vi "Versioned Load.vi"(10 "path":path) -> (0 "Reversals":T10, 1 "Trajectory Data":T1, 2 "Zero V":bool, 3 "Commands out":cluster{"Time (s)":dbl, T8, bool}[](array[cluster]), 4 "Fields":T7 {"Overrides"."Angle Override" step=5.0; "Overrides"."Velocity Override" step=5.0; "Overrides"."Angular Override" step=5.0; "Angular Limits"."Jerk (deg/s^3)" min=0.0 step=1.0; "Angular Limits"."Accel (deg/s^2)" min=0.0; "Angular Limits"."Velocity (deg/s)" min=0.0}, 5 "Points out":cluster{"x":dbl, "y":dbl, "th":dbl}[](array[cluster]), 6 "Trajectory Meta":cluster{"Drive Type":T3, "Path Type":T4}, 7 "Overall":cluster{"Time (s)":dbl, "Distance (ft)":dbl})   [LabVIEW 2025]
uses:
  bordeaux-main/Bordeaux/Types/Single Cmd Info.ctl
  <vilib>/picture/picture.llb/imagedata.ctl
  bordeaux-main/Bordeaux/Types/Overrides.ctl
  bordeaux-main/Bordeaux/Types/Angluar Limits.ctl
  bordeaux-main/Bordeaux/Types/Drive Type.ctl
  bordeaux-main/Bordeaux/Types/Path Type.ctl
  bordeaux-main/Bordeaux/Types/Trajectory Data.ctl
  bordeaux-main/Bordeaux/Types/Segment Type.ctl
  bordeaux-main/Bordeaux/Types/Availible Command systems for auto.ctl
  bordeaux-main/Bordeaux/Types/Limits.ctl
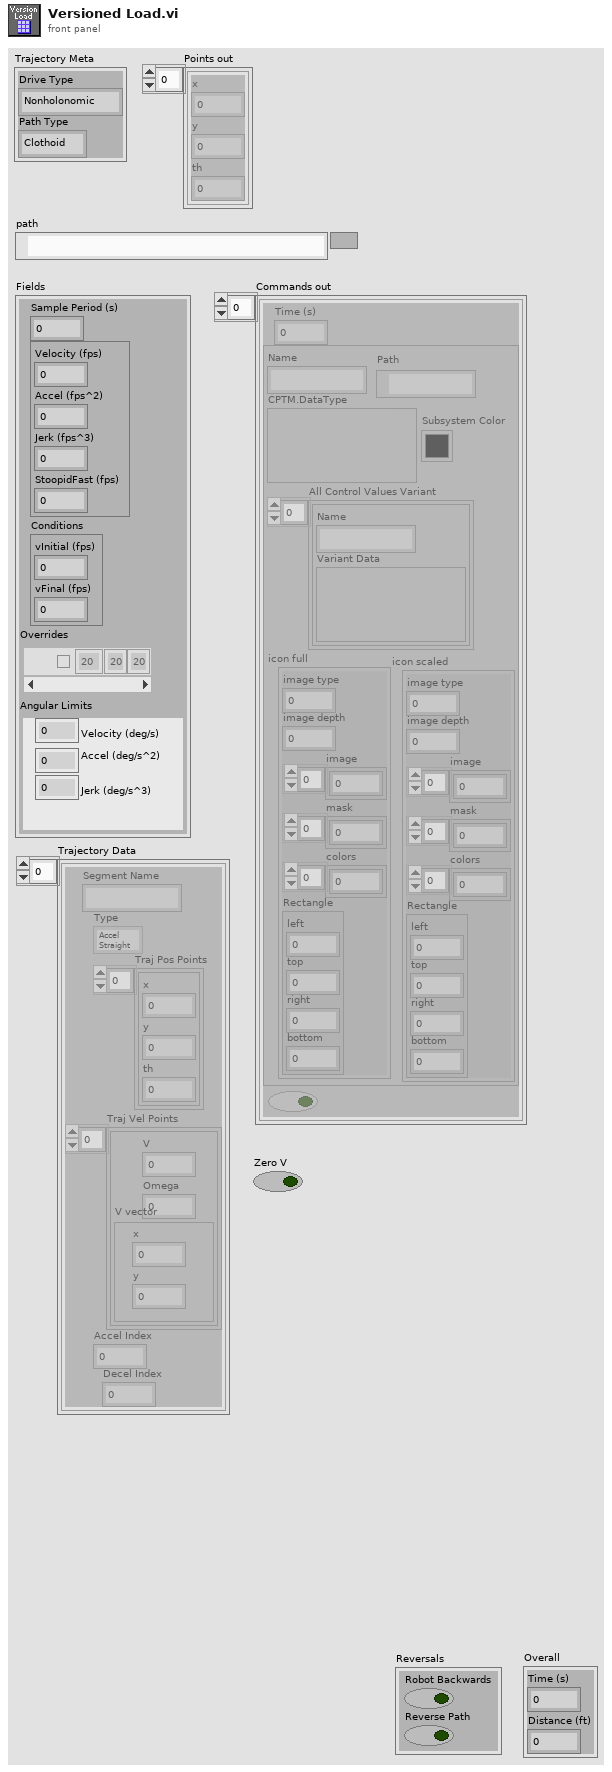
[diagram p1: front panel]
types:
  T1 = typedef "Trajectory Data.ctl" = cluster{"Segment Name":string, "Type":T2, "Traj Pos Points":cluster{"x":dbl, "y":dbl, "th":dbl}[], "Traj Vel Points":cluster{"V":dbl, "Omega":dbl, "V vector":cluster{"y":dbl, "x":dbl}}[], "Accel Index":i32, "Decel Index":i32}[]
  T2 = typedef "Segment Type.ctl" = enum16{"Accel Straight", "Const Straight", "Blend", "Circle", "Bezier"}
  T3 = typedef "Drive Type.ctl" = enum16{"Nonholonomic", "Holonomic"}
  T4 = typedef "Path Type.ctl" = enum16{"Clothoid", "Bezier"}
  T5 = typedef "Overrides.ctl" = cluster{"Count":string, "Angular Override":dbl, "Enabled?":bool, "Velocity Override":dbl, "Angle Override":dbl}[]
  T6 = typedef "Angluar Limits.ctl" = cluster{"Velocity (deg/s)":dbl, "Accel (deg/s^2)":dbl, "Jerk (deg/s^3)":dbl}
  T7 = cluster{"Sample Period (s)":dbl, cluster{"Velocity (fps)":dbl, "Accel (fps^2)":dbl, "Jerk (fps^3)":dbl, "StoopidFast (fps)":dbl}, "Conditions":cluster{"vInitial (fps)":dbl, "vFinal (fps)":dbl}, "Overrides":T5, "Angular Limits":T6}
  T8 = typedef "Single Cmd Info.ctl" = cluster{"Name":string, "CPTM.DataType":variant, "All Control Values Variant":cluster{"Name":string, "Variant Data":variant}[], "icon full":T9, "icon scaled":T9, "Path":path, "Subsystem Color":u32}
  T9 = typedef "imagedata.ctl" = cluster{"image type":i32, "image depth":i32, "image":u8[], "mask":u8[], "colors":u32[], "Rectangle":cluster{"left":i16, "top":i16, "right":i16, "bottom":i16}}
  T10 = cluster{"Robot Backwards":bool, "Reverse Path":bool}
  T11 = cluster{"Sample Period (s)":dbl, "Limits 2":cluster{"Velocity (fps)":dbl, "Acceleration (fps^2)":dbl, "Jerk (fps^3)":dbl}, "Conditions":cluster{"vInitial (fps)":dbl, "vFinal (fps)":dbl}, " Acceleration Overrides":cluster{"Angular \nAccelerations":dbl[], "Accel Override Bools":bool[]}}
  T12 = cluster{"Velocity":dbl, "Sample Time":dbl, "Accel":dbl}
  T13 = cluster{"Sample Period (s)":dbl, "Limits":cluster{"Velocity (fps)":dbl, "Acceleration (fps^2)":dbl, "Jerk (fps^3)":dbl}, "Conditions":cluster{"vInitial (fps)":dbl, "vFinal (fps)":dbl}}
  T14 = cluster{"Sample Period (s)":dbl, "Limits":cluster{"Velocity (fps)":dbl, "Acceleration (fps^2)":dbl, "Jerk (fps^3)":dbl}, "Conditions":cluster{"vInitial (fps)":dbl, "vFinal (fps)":dbl}, "Min Rads":dbl[]}
  T15 = typedef "Availible Command systems for auto.ctl" = u16
  T16 = cluster{"Time into Path":dbl, "System":T15, "Item Selected?":bool, "System Selection":T15}[]
  T17 = cluster{"Sample Period (s)":dbl, "Limits 2":cluster{"Velocity (fps)":dbl, "Acceleration (fps^2)":dbl, "Jerk (fps^3)":dbl, "Stoopid Fast":dbl}, "Conditions":cluster{"vInitial (fps)":dbl, "vFinal (fps)":dbl}, " Acceleration Overrides":cluster{"Angular \nAccelerations":dbl[], "Accel Override Bools":bool[]}}
  T18 = cluster{"Sample Period (s)":dbl, "Limits":cluster{"Velocity (fps)":dbl, "Accel (fps^2)":dbl, "Turn Accel (fps^2)":dbl, "Jerk (fps^3)":dbl}, "Conditions":cluster{"vInitial (fps)":dbl, "vFinal (fps)":dbl}, cluster{dbl[], bool[]}}
  T19 = cluster{"Reverse Path":bool, "Robot Backwards":bool}
  T20 = typedef "Limits.ctl" = cluster{"Velocity (fps)":dbl, "Accel (fps^2)":dbl, "Jerk (fps^3)":dbl, "StoopidFast (fps)":dbl}
  T21 = cluster{"Sample Period (s)":dbl, "Limits":T20, "Conditions":cluster{"vInitial (fps)":dbl, "vFinal (fps)":dbl}, "Overrides":T5, "Angular Limits":T6}
  T22 = cluster{"Velocity":dbl, "Accel":dbl, "Accel":dbl, "Velocity":dbl}
  T23 = cluster{"Velocity (fps)":dbl, "Acceleration (fps^2)":dbl, "Jerk (fps^3)":dbl}
  T24 = cluster{"vInitial (fps)":dbl, "vFinal (fps)":dbl}
  T25 = cluster{"Velocity (fps)":dbl, "Acceleration (fps^2)":dbl, "Jerk (fps^3)":dbl, "Velocity (fps)":dbl}
  T26 = cluster{string, "Angular Multiplier":dbl, bool, "Velocity (fps)":dbl, "Velocity (fps)":dbl}
  T27 = cluster{"Angular \nAccelerations":dbl[], "Accel Override Bools":bool[]}
  T28 = cluster{"Velocity (fps)":dbl, "Acceleration (fps^2)":dbl, "Jerk (fps^3)":dbl, "Stoopid Fast":dbl}
  T29 = cluster{"Velocity (fps)":dbl, "Accel (fps^2)":dbl, "Turn Accel (fps^2)":dbl, "Jerk (fps^3)":dbl}
  T30 = cluster{"Velocity (fps)":dbl, "Accel (fps^2)":dbl, "Jerk (fps^3)":dbl, "StoopidFast (fps)":dbl}
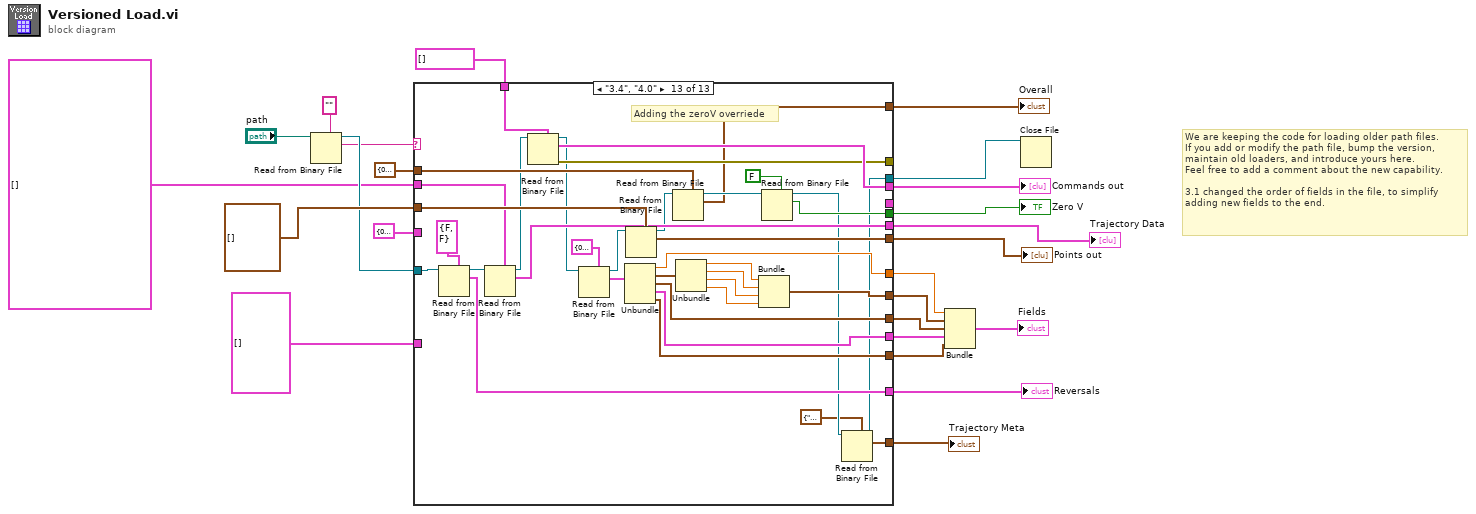
[diagram p0: block diagram]
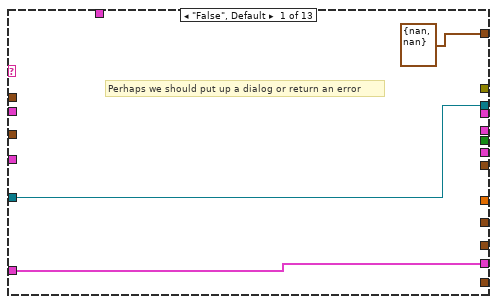
[diagram p2: hidden frame]
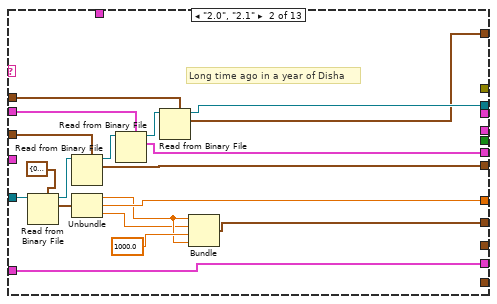
[diagram p3: hidden frame]
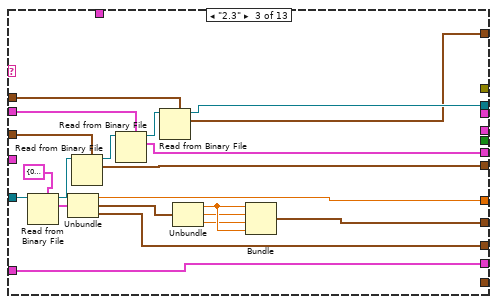
[diagram p4: hidden frame]
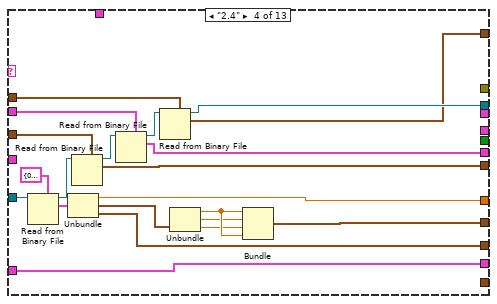
[diagram p5: hidden frame]
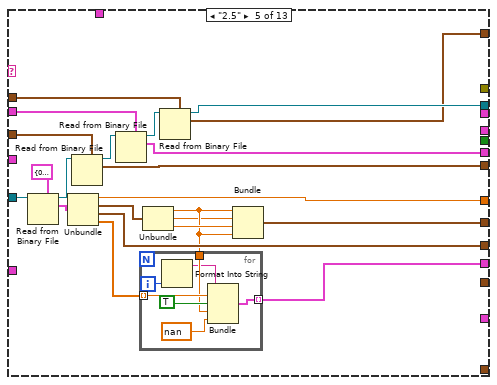
[diagram p6: hidden frame]
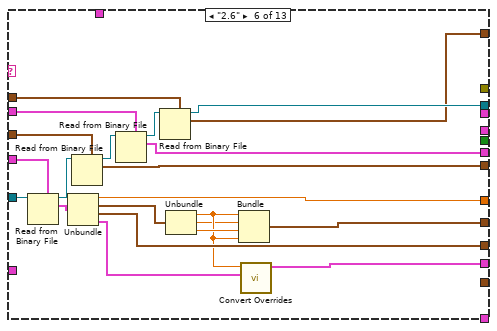
[diagram p7: hidden frame]
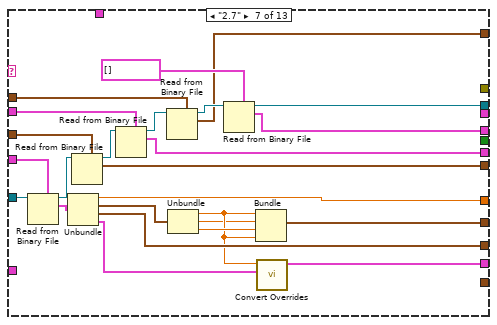
[diagram p8: hidden frame]
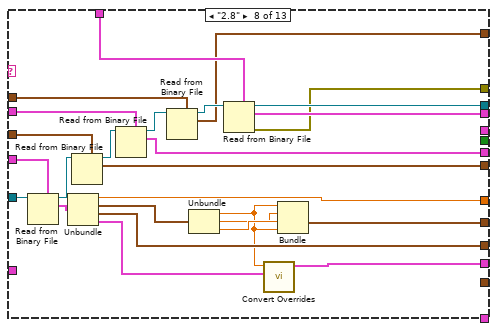
[diagram p9: hidden frame]
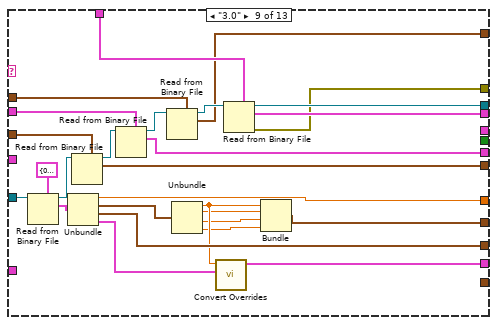
[diagram p10: hidden frame]
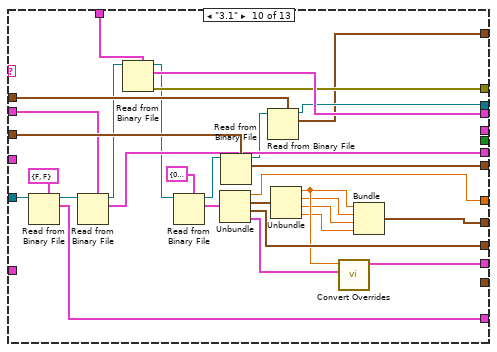
[diagram p11: hidden frame]
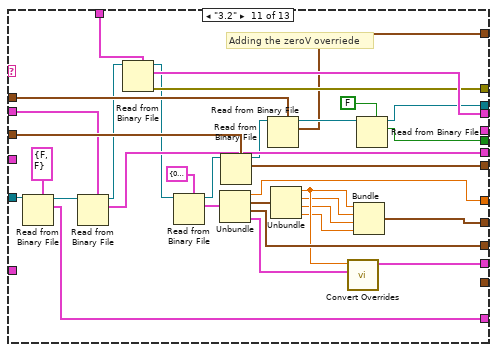
[diagram p12: hidden frame]
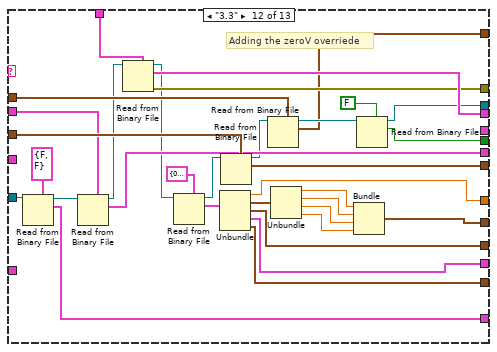
[diagram p13: hidden frame]
diagram:
  # "We are keeping the code for loading older path files.\nIf you add or modify the path file, bump the version,\nmaintain old loaders, and introduce yours here.\nFeel free to add a comment about the new capability.\n\n3.1 changed the order of fields in the file, to simplify\nadding new fields to the end."
  n1 = Read from Binary File(5:"" ("String"), 11:"path") -> (2:w7:string, 3:w8:refnum<file>)  [unwired: 4 in, 2 out]
  n2 = case shown="\"3.4\", \"4.0\"" w7 {
    tunnel: w8 -> [w27 w45 w66 w87 w109 w138 w163 w189 w216 w236 w269 w302 w338]
    tunnel: cluster{"x":dbl, "y":dbl, "th":dbl}[] [] ("Points in") -> [_ w43 w64 w85 w107 w136 w161 w187 w214 w245 w278 w311 w347]
    tunnel: [_ w42 w63 w84 w106 w135 w160 w186 w213 w244 w277 w310 w346] -> w14
    tunnel: T1 [] ("Trajectory Data") -> [_ w41 w62 w83 w105 w134 w159 w185 w212 w243 w276 w309 w345]
    tunnel: cluster{"Time (s)":dbl, "Distance (ft)":dbl} {"Time (s)"=0.0, "Distance (ft)"=0.0} ("Cluster 4") -> [_ w39 w60 w81 w103 w132 w157 w183 w210 w242 w275 w308 w344]
    tunnel: [w27 w37 w58 w79 w101 w130 w151 w177 w204 w232 w251 w287 w315] -> w10
    tunnel: [_ w35 w57 w78 w100 w129 w155 w181 w208 w219 w253 w289 w325] -> w21
    tunnel: [_ w31 w51 w71 w94 w124 w145 w172 w192 w224 w258 w294 w330] -> w22
    tunnel: [_ _ w56 w77 w99 w128 w154 w180 w207 w241 w274 w307 w343] -> w23
    tunnel: [w26 w30 w50 w70 w93 w122 w142 w169 w198 w228 w262 w282 w319] -> w24
    tunnel: [_ w33 w54 w75 w97 w127 w153 w179 w206 w240 w273 w306 w342] -> w13
    tunnel: [_ _ _ _ _ _ w150 _ _ _ _ _ _] -> _
    tunnel: cluster{"Time (s)":dbl, T8, bool}[] [] ("Commands in") -> [_ _ _ _ _ _ _ w176 w203 w239 w272 w305 w341]
    tunnel: [_ _ _ _ _ _ _ w175 w202 w238 w271 w304 w340] -> w16
    tunnel: [_ _ _ _ _ _ _ w174 w201 w237 w270 w303 w339] -> _
    tunnel: T11 {"Sample Period (s)"=0.0, "Limits 2"={"Velocity (fps)"=0.0, "Acceleration (fps^2)"=0.0, "Jerk (fps^3)"=0.0}, "Conditions"={"vInitial (fps)"=0.0, "vFinal (fps)"=0.0}, " Acceleration Overrides"={"Angular \nAccelerations"=[], "Accel Override Bools"=[]}} ("Cluster") -> [_ _ _ _ _ w126 w148 w170 _ _ _ _ _]
    tunnel: [_ _ _ _ _ _ _ _ _ w227 w261 w296 w332] -> w18
    tunnel: T5 [] ("Overrides") -> [w26 w30 w50 w70 _ _ _ _ _ _ _ _ _]
    tunnel: [_ _ _ _ _ _ _ _ _ _ w249 w285 w322] -> w19
    tunnel: [cluster{"Time (s)":dbl, "Distance (ft)":dbl} {"Time (s)"=nan, "Distance (ft)"=nan} ("Cluster 4") w28 w47 w68 w89 w118 w140 w165 w191 w218 w248 w284 w321] -> w5
    tunnel: [_ _ _ _ _ _ _ _ _ _ _ w281 w318] -> w2
    tunnel: [_ _ _ _ _ _ _ _ _ _ _ _ w314] -> w1
    frame "False", Default {
      # "Perhaps we should put up a dialog or return an error"
    }
    frame "2.0", "2.1" {
      # "Long time ago in a year of Disha"
      n3 = Read from Binary File(5:T12 {"Velocity"=0.0, "Sample Time"=0.0, "Accel"=0.0}, 11:w45) -> (2:w46:T12, 3:w44:refnum<file>)  [unwired: 4 in, 2 out]
      n4 = Read from Binary File(5:w43, 11:w44) -> (2:w42:cluster{"x":dbl, "y":dbl, "th":dbl}[], 3:w40:refnum<file>)  [unwired: 4 in, 2 out]
      n5 = Unbundle(w46) -> ("Velocity"=w32:dbl, "Sample Time"=w35:dbl, "Accel"=w29:dbl)
      n6 = Read from Binary File(5:w41, 11:w40) -> (2:w33:T1, 3:w38:refnum<file>)  [unwired: 4 in, 2 out]
      n7 = Read from Binary File(5:w39, 11:w38) -> (2:w28:cluster{"Time (s)":dbl, "Distance (ft)":dbl}, 3:w37:refnum<file>)  [unwired: 4 in, 2 out]
      n8 = Bundle("Velocity"=w32, "Accel"=w29, "Accel"=1000.0, "Velocity"=w32) -> (w31:T22)  [unwired: 1 in]
    }
    frame "2.3" {
      n9 = Read from Binary File(5:T13 {"Sample Period (s)"=0.0, "Limits"={"Velocity (fps)"=0.0, "Acceleration (fps^2)"=0.0, "Jerk (fps^3)"=0.0}, "Conditions"={"vInitial (fps)"=0.0, "vFinal (fps)"=0.0}}, 11:w66) -> (2:w67:T13, 3:w65:refnum<file>)  [unwired: 4 in, 2 out]
      n10 = Unbundle(w67) -> ("Sample Period (s)"=w57:dbl, "Limits"=w48:T23, "Conditions"=w56:T24)
      n11 = Read from Binary File(5:w64, 11:w65) -> (2:w63:cluster{"x":dbl, "y":dbl, "th":dbl}[], 3:w61:refnum<file>)  [unwired: 4 in, 2 out]
      n12 = Read from Binary File(5:w62, 11:w61) -> (2:w54:T1, 3:w59:refnum<file>)  [unwired: 4 in, 2 out]
      n13 = Read from Binary File(5:w60, 11:w59) -> (2:w47:cluster{"Time (s)":dbl, "Distance (ft)":dbl}, 3:w58:refnum<file>)  [unwired: 4 in, 2 out]
      n14 = Unbundle(w48) -> ("Velocity (fps)"=w53:dbl, "Acceleration (fps^2)"=w49:dbl, "Jerk (fps^3)"=w52:dbl)
      n15 = Bundle("Velocity (fps)"=w53, "Acceleration (fps^2)"=w49, "Jerk (fps^3)"=w52, "Velocity (fps)"=w53) -> (w51:T25)  [unwired: 1 in]
    }
    frame "2.4" {
      n16 = Read from Binary File(5:T13 {"Sample Period (s)"=0.0, "Limits"={"Velocity (fps)"=0.0, "Acceleration (fps^2)"=0.0, "Jerk (fps^3)"=0.0}, "Conditions"={"vInitial (fps)"=0.0, "vFinal (fps)"=0.0}}, 11:w87) -> (2:w88:T13, 3:w86:refnum<file>)  [unwired: 4 in, 2 out]
      n17 = Unbundle(w88) -> ("Sample Period (s)"=w78:dbl, "Limits"=w72:T23, "Conditions"=w77:T24)
      n18 = Read from Binary File(5:w85, 11:w86) -> (2:w84:cluster{"x":dbl, "y":dbl, "th":dbl}[], 3:w82:refnum<file>)  [unwired: 4 in, 2 out]
      n19 = Read from Binary File(5:w83, 11:w82) -> (2:w75:T1, 3:w80:refnum<file>)  [unwired: 4 in, 2 out]
      n20 = Read from Binary File(5:w81, 11:w80) -> (2:w68:cluster{"Time (s)":dbl, "Distance (ft)":dbl}, 3:w79:refnum<file>)  [unwired: 4 in, 2 out]
      n21 = Unbundle(w72) -> ("Velocity (fps)"=w74:dbl, "Acceleration (fps^2)"=w69:dbl, "Jerk (fps^3)"=w73:dbl)
      n22 = Bundle("Velocity (fps)"=w74, "Acceleration (fps^2)"=w69, "Jerk (fps^3)"=w73, "Velocity (fps)"=w74) -> (w71:T25)  [unwired: 1 in]
    }
    frame "2.5" {
      n23 = Read from Binary File(5:T14 {"Sample Period (s)"=0.0, "Limits"={"Velocity (fps)"=0.0, "Acceleration (fps^2)"=0.0, "Jerk (fps^3)"=0.0}, "Conditions"={"vInitial (fps)"=0.0, "vFinal (fps)"=0.0}, "Min Rads"=[20.0, 20.0, 20.0, 20.0, 20.0]}, 11:w109) -> (2:w110:T14, 3:w108:refnum<file>)  [unwired: 4 in, 2 out]
      n24 = Unbundle(w110) -> ("Sample Period (s)"=w100:dbl, "Limits"=w95:T23, "Conditions"=w99:T24, "Min Rads"=w92:dbl[])
      n25 = Read from Binary File(5:w107, 11:w108) -> (2:w106:cluster{"x":dbl, "y":dbl, "th":dbl}[], 3:w104:refnum<file>)  [unwired: 4 in, 2 out]
      n26 = Read from Binary File(5:w105, 11:w104) -> (2:w97:T1, 3:w102:refnum<file>)  [unwired: 4 in, 2 out]
      n27 = Unbundle(w95) -> ("Velocity (fps)"=w91:dbl, "Acceleration (fps^2)"=w90:dbl, "Jerk (fps^3)"=w96:dbl)
      n28 = for {
        tunnel: [w116] -> w93 mode=indexing
        tunnel: w92 -> [w115] mode=indexing
        tunnel: w91 -> [w114]
        i -> [w113]
        n29 = Format Into String(w113) -> (resulting string=w112:string)  [unwired: 3 in, 1 out]
        n30 = Bundle(w112, "Angular Multiplier"=w115, TRUE, "Velocity (fps)"=w114, "Velocity (fps)"=nan) -> (w116:T26)  [unwired: 1 in]
      }
      n31 = Read from Binary File(5:w103, 11:w102) -> (2:w89:cluster{"Time (s)":dbl, "Distance (ft)":dbl}, 3:w101:refnum<file>)  [unwired: 4 in, 2 out]
      n32 = Bundle("Velocity (fps)"=w91, "Acceleration (fps^2)"=w90, "Jerk (fps^3)"=w96, "Velocity (fps)"=w91) -> (w94:T25)  [unwired: 1 in]
    }
    frame "2.6" {
      n33 = Read from Binary File(5:w126, 11:w138) -> (2:w139:T11, 3:w137:refnum<file>)  [unwired: 4 in, 2 out]
      n34 = Unbundle(w139) -> ("Sample Period (s)"=w129:dbl, "Limits 2"=w123:T23, "Conditions"=w128:T24, "Acceleration Overrides"=w120:T27)
      n35 = Read from Binary File(5:w136, 11:w137) -> (2:w135:cluster{"x":dbl, "y":dbl, "th":dbl}[], 3:w133:refnum<file>)  [unwired: 4 in, 2 out]
      n36 = Read from Binary File(5:w134, 11:w133) -> (2:w127:T1, 3:w131:refnum<file>)  [unwired: 4 in, 2 out]
      n37 = Read from Binary File(5:w132, 11:w131) -> (2:w118:cluster{"Time (s)":dbl, "Distance (ft)":dbl}, 3:w130:refnum<file>)  [unwired: 4 in, 2 out]
      n38 = Unbundle(w123) -> ("Velocity (fps)"=w121:dbl, "Acceleration (fps^2)"=w119:dbl, "Jerk (fps^3)"=w125:dbl)
      n39 = Bundle("Velocity (fps)"=w121, "Acceleration (fps^2)"=w119, "Jerk (fps^3)"=w125, "Velocity (fps)"=w121) -> (w124:T25)  [unwired: 1 in]
      n40 = call "Convert Overrides.vi"("Cluster"=w120, "Velocity (fps)"=w121) -> ("Overrides"=w122:T5)  [unwired: 9 in]
    }
    frame "2.7" {
      n41 = Read from Binary File(5:w148, 11:w163) -> (2:w164:T11, 3:w162:refnum<file>)  [unwired: 4 in, 2 out]
      n42 = Unbundle(w164) -> ("Sample Period (s)"=w155:dbl, "Limits 2"=w146:T23, "Conditions"=w154:T24, "Acceleration Overrides"=w143:T27)
      n43 = Read from Binary File(5:w161, 11:w162) -> (2:w160:cluster{"x":dbl, "y":dbl, "th":dbl}[], 3:w158:refnum<file>)  [unwired: 4 in, 2 out]
      n44 = Read from Binary File(5:w159, 11:w158) -> (2:w153:T1, 3:w156:refnum<file>)  [unwired: 4 in, 2 out]
      n45 = Read from Binary File(5:w157, 11:w156) -> (2:w140:cluster{"Time (s)":dbl, "Distance (ft)":dbl}, 3:w152:refnum<file>)  [unwired: 4 in, 2 out]
      n46 = Unbundle(w146) -> ("Velocity (fps)"=w144:dbl, "Acceleration (fps^2)"=w141:dbl, "Jerk (fps^3)"=w147:dbl)
      n47 = Read from Binary File(5:T16 [] ("Commands"), 11:w152) -> (2:w150:T16, 3:w151:refnum<file>)  [unwired: 4 in, 2 out]
      n48 = Bundle("Velocity (fps)"=w144, "Acceleration (fps^2)"=w141, "Jerk (fps^3)"=w147, "Velocity (fps)"=w144) -> (w145:T25)  [unwired: 1 in]
      n49 = call "Convert Overrides.vi"("Cluster"=w143, "Velocity (fps)"=w144) -> ("Overrides"=w142:T5)  [unwired: 9 in]
    }
    frame "2.8" {
      n50 = Read from Binary File(5:w170, 11:w189) -> (2:w190:T11, 3:w188:refnum<file>)  [unwired: 4 in, 2 out]
      n51 = Unbundle(w190) -> ("Sample Period (s)"=w181:dbl, "Limits 2"=w173:T23, "Conditions"=w180:T24, "Acceleration Overrides"=w167:T27)
      n52 = Read from Binary File(5:w187, 11:w188) -> (2:w186:cluster{"x":dbl, "y":dbl, "th":dbl}[], 3:w184:refnum<file>)  [unwired: 4 in, 2 out]
      n53 = Read from Binary File(5:w185, 11:w184) -> (2:w179:T1, 3:w182:refnum<file>)  [unwired: 4 in, 2 out]
      n54 = Read from Binary File(5:w183, 11:w182) -> (2:w165:cluster{"Time (s)":dbl, "Distance (ft)":dbl}, 3:w178:refnum<file>)  [unwired: 4 in, 2 out]
      n55 = Unbundle(w173) -> ("Velocity (fps)"=w168:dbl, "Acceleration (fps^2)"=w166:dbl, "Jerk (fps^3)"=w171:dbl)
      n56 = Read from Binary File(5:w176, 11:w178) -> (0:w174:errorcluster, 2:w175:cluster{"Time (s)":dbl, T8, bool}[], 3:w177:refnum<file>)  [unwired: 4 in, 1 out]
      n57 = call "Convert Overrides.vi"("Cluster"=w167, "Velocity (fps)"=w168) -> ("Overrides"=w169:T5)  [unwired: 9 in]
      n58 = Bundle("Velocity (fps)"=w168, "Acceleration (fps^2)"=w166, "Jerk (fps^3)"=w171, "Velocity (fps)"=w168) -> (w172:T25)  [unwired: 1 in]
    }
    frame "3.0" {
      n59 = Read from Binary File(5:T17 {"Sample Period (s)"=0.0, "Limits 2"={"Velocity (fps)"=0.0, "Acceleration (fps^2)"=0.0, "Jerk (fps^3)"=0.0, "Stoopid Fast"=0.0}, "Conditions"={"vInitial (fps)"=0.0, "vFinal (fps)"=0.0}, " Acceleration Overrides"={"Angular \nAccelerations"=[], "Accel Override Bools"=[]}} ("Cluster"), 11:w216) -> (2:w217:T17, 3:w215:refnum<file>)  [unwired: 4 in, 2 out]
      n60 = Unbundle(w217) -> ("Sample Period (s)"=w208:dbl, "Limits 2"=w193:T28, "Conditions"=w207:T24, "Acceleration Overrides"=w199:T27)
      n61 = Read from Binary File(5:w214, 11:w215) -> (2:w213:cluster{"x":dbl, "y":dbl, "th":dbl}[], 3:w211:refnum<file>)  [unwired: 4 in, 2 out]
      n62 = Read from Binary File(5:w212, 11:w211) -> (2:w206:T1, 3:w209:refnum<file>)  [unwired: 4 in, 2 out]
      n63 = Read from Binary File(5:w210, 11:w209) -> (2:w191:cluster{"Time (s)":dbl, "Distance (ft)":dbl}, 3:w205:refnum<file>)  [unwired: 4 in, 2 out]
      n64 = Unbundle(w193) -> ("Velocity (fps)"=w197:dbl, "Acceleration (fps^2)"=w196:dbl, "Jerk (fps^3)"=w195:dbl, "Stoopid Fast"=w194:dbl)
      n65 = call "Convert Overrides.vi"("Cluster"=w199, "Velocity (fps)"=w197) -> ("Overrides"=w198:T5)  [unwired: 9 in]
      n66 = Read from Binary File(5:w203, 11:w205) -> (0:w201:errorcluster, 2:w202:cluster{"Time (s)":dbl, T8, bool}[], 3:w204:refnum<file>)  [unwired: 4 in, 1 out]
      n67 = Bundle("Velocity (fps)"=w197, "Acceleration (fps^2)"=w196, "Jerk (fps^3)"=w195, "Stoopid Fast"=w194) -> (w192:T28)  [unwired: 1 in]
    }
    frame "3.1" {
      n68 = Read from Binary File(5:T19 {"Reverse Path"=FALSE, "Robot Backwards"=FALSE} ("Cluster"), 11:w236) -> (2:w227:T19, 3:w233:refnum<file>)  [unwired: 4 in, 2 out]
      n69 = Read from Binary File(5:w243, 11:w233) -> (2:w240:T1, 3:w231:refnum<file>)  [unwired: 4 in, 2 out]
      n70 = Read from Binary File(5:w239, 11:w231) -> (0:w237:errorcluster, 2:w238:cluster{"Time (s)":dbl, T8, bool}[], 3:w230:refnum<file>)  [unwired: 4 in, 1 out]
      n71 = Read from Binary File(5:T18 {"Sample Period (s)"=0.0, "Limits"={"Velocity (fps)"=0.0, "Accel (fps^2)"=0.0, "Turn Accel (fps^2)"=15.0, "Jerk (fps^3)"=0.0}, "Conditions"={"vInitial (fps)"=0.0, "vFinal (fps)"=0.0}, {[], []}} ("Cluster 2"), 11:w230) -> (2:w247:T18, 3:w246:refnum<file>)  [unwired: 4 in, 2 out]
      n72 = Unbundle(w247) -> ("Sample Period (s)"=w219:dbl, "Limits"=w226:T29, "Conditions"=w241:T24, w229:cluster{dbl[], bool[]})
      n73 = Read from Binary File(5:w245, 11:w246) -> (2:w244:cluster{"x":dbl, "y":dbl, "th":dbl}[], 3:w234:refnum<file>)  [unwired: 4 in, 2 out]
      n74 = Read from Binary File(5:w242, 11:w234) -> (2:w218:cluster{"Time (s)":dbl, "Distance (ft)":dbl}, 3:w232:refnum<file>)  [unwired: 4 in, 2 out]
      n75 = Unbundle(w226) -> ("Velocity (fps)"=w223:dbl, "Accel (fps^2)"=w222:dbl, "Turn Accel (fps^2)"=w221:dbl, "Jerk (fps^3)"=w220:dbl)
      n76 = call "Convert Overrides.vi"("Cluster"=w229, "Velocity (fps)"=w223) -> ("Overrides"=w228:T5)  [unwired: 9 in]
      n77 = Bundle("Velocity (fps)"=w223, "Accel (fps^2)"=w222, "Turn Accel (fps^2)"=w221, "Jerk (fps^3)"=w220) -> (w224:T29)  [unwired: 1 in]
    }
    frame "3.2" {
      # "Adding the zeroV overriede"
      n78 = Read from Binary File(5:T10 {"Robot Backwards"=FALSE, "Reverse Path"=FALSE} ("Cluster"), 11:w269) -> (2:w261:T10, 3:w266:refnum<file>)  [unwired: 4 in, 2 out]
      n79 = Read from Binary File(5:w276, 11:w266) -> (2:w273:T1, 3:w265:refnum<file>)  [unwired: 4 in, 2 out]
      n80 = Read from Binary File(5:w272, 11:w265) -> (0:w270:errorcluster, 2:w271:cluster{"Time (s)":dbl, T8, bool}[], 3:w264:refnum<file>)  [unwired: 4 in, 1 out]
      n81 = Read from Binary File(5:T18 {"Sample Period (s)"=0.0, "Limits"={"Velocity (fps)"=0.0, "Accel (fps^2)"=0.0, "Turn Accel (fps^2)"=15.0, "Jerk (fps^3)"=0.0}, "Conditions"={"vInitial (fps)"=0.0, "vFinal (fps)"=0.0}, {[], []}} ("Cluster 2"), 11:w264) -> (2:w280:T18, 3:w279:refnum<file>)  [unwired: 4 in, 2 out]
      n82 = Unbundle(w280) -> ("Sample Period (s)"=w253:dbl, "Limits"=w260:T29, "Conditions"=w274:T24, w263:cluster{dbl[], bool[]})
      n83 = Read from Binary File(5:w278, 11:w279) -> (2:w277:cluster{"x":dbl, "y":dbl, "th":dbl}[], 3:w267:refnum<file>)  [unwired: 4 in, 2 out]
      n84 = Read from Binary File(5:w275, 11:w267) -> (2:w248:cluster{"Time (s)":dbl, "Distance (ft)":dbl}, 3:w252:refnum<file>)  [unwired: 4 in, 2 out]
      n85 = Unbundle(w260) -> ("Velocity (fps)"=w257:dbl, "Accel (fps^2)"=w256:dbl, "Turn Accel (fps^2)"=w255:dbl, "Jerk (fps^3)"=w254:dbl)
      n86 = call "Convert Overrides.vi"("Cluster"=w263, "Velocity (fps)"=w257) -> ("Overrides"=w262:T5)  [unwired: 9 in]
      n87 = Bundle("Velocity (fps)"=w257, "Accel (fps^2)"=w256, "Turn Accel (fps^2)"=w255, "Jerk (fps^3)"=w254) -> (w258:T29)  [unwired: 1 in]
      n88 = Read from Binary File(5:FALSE, 11:w252) -> (2:w249:bool, 3:w251:refnum<file>)  [unwired: 4 in, 2 out]
    }
    frame "3.3" {
      # "Adding the zeroV overriede"
      n89 = Read from Binary File(5:T10 {"Robot Backwards"=FALSE, "Reverse Path"=FALSE} ("Cluster"), 11:w302) -> (2:w296:T10, 3:w299:refnum<file>)  [unwired: 4 in, 2 out]
      n90 = Read from Binary File(5:w309, 11:w299) -> (2:w306:T1, 3:w298:refnum<file>)  [unwired: 4 in, 2 out]
      n91 = Read from Binary File(5:w305, 11:w298) -> (0:w303:errorcluster, 2:w304:cluster{"Time (s)":dbl, T8, bool}[], 3:w297:refnum<file>)  [unwired: 4 in, 1 out]
      n92 = Read from Binary File(5:T21 {"Sample Period (s)"=0.0, "Limits"={"Velocity (fps)"=0.0, "Accel (fps^2)"=0.0, "Jerk (fps^3)"=0.0, "StoopidFast (fps)"=0.0}, "Conditions"={"vInitial (fps)"=0.0, "vFinal (fps)"=0.0}, "Overrides"=[], "Angular Limits"={"Velocity (deg/s)"=0.0, "Accel (deg/s^2)"=0.0, "Jerk (deg/s^3)"=0.0}} ("output cluster"), 11:w297) -> (2:w313:T21, 3:w312:refnum<file>)  [unwired: 4 in, 2 out]
      n93 = Unbundle(w313) -> ("Sample Period (s)"=w289:dbl, "Limits"=w295:T20, "Conditions"=w307:T24, "Overrides"=w282:T5, "Angular Limits"=w281:T6)
      n94 = Read from Binary File(5:w311, 11:w312) -> (2:w310:cluster{"x":dbl, "y":dbl, "th":dbl}[], 3:w300:refnum<file>)  [unwired: 4 in, 2 out]
      n95 = Read from Binary File(5:w308, 11:w300) -> (2:w284:cluster{"Time (s)":dbl, "Distance (ft)":dbl}, 3:w288:refnum<file>)  [unwired: 4 in, 2 out]
      n96 = Unbundle(w295) -> ("Velocity (fps)"=w293:dbl, "Accel (fps^2)"=w292:dbl, "Jerk (fps^3)"=w291:dbl, "StoopidFast (fps)"=w290:dbl)
      n97 = Bundle("Velocity (fps)"=w293, "Accel (fps^2)"=w292, "Jerk (fps^3)"=w291, "StoopidFast (fps)"=w290) -> (w294:T30)  [unwired: 1 in]
      n98 = Read from Binary File(5:FALSE, 11:w288) -> (2:w285:bool, 3:w287:refnum<file>)  [unwired: 4 in, 2 out]
    }
    frame "3.4", "4.0" {
      # "Adding the zeroV overriede"
      n99 = Read from Binary File(5:T10 {"Robot Backwards"=FALSE, "Reverse Path"=FALSE} ("Cluster"), 11:w338) -> (2:w332:T10, 3:w335:refnum<file>)  [unwired: 4 in, 2 out]
      n100 = Read from Binary File(5:w345, 11:w335) -> (2:w342:T1, 3:w334:refnum<file>)  [unwired: 4 in, 2 out]
      n101 = Read from Binary File(5:w341, 11:w334) -> (0:w339:errorcluster, 2:w340:cluster{"Time (s)":dbl, T8, bool}[], 3:w333:refnum<file>)  [unwired: 4 in, 1 out]
      n102 = Read from Binary File(5:T21 {"Sample Period (s)"=0.0, "Limits"={"Velocity (fps)"=0.0, "Accel (fps^2)"=0.0, "Jerk (fps^3)"=0.0, "StoopidFast (fps)"=0.0}, "Conditions"={"vInitial (fps)"=0.0, "vFinal (fps)"=0.0}, "Overrides"=[], "Angular Limits"={"Velocity (deg/s)"=0.0, "Accel (deg/s^2)"=0.0, "Jerk (deg/s^3)"=0.0}} ("output cluster"), 11:w333) -> (2:w349:T21, 3:w348:refnum<file>)  [unwired: 4 in, 2 out]
      n103 = Unbundle(w349) -> ("Sample Period (s)"=w325:dbl, "Limits"=w331:T20, "Conditions"=w343:T24, "Overrides"=w319:T5, "Angular Limits"=w318:T6)
      n104 = Read from Binary File(5:w347, 11:w348) -> (2:w346:cluster{"x":dbl, "y":dbl, "th":dbl}[], 3:w336:refnum<file>)  [unwired: 4 in, 2 out]
      n105 = Read from Binary File(5:w344, 11:w336) -> (2:w321:cluster{"Time (s)":dbl, "Distance (ft)":dbl}, 3:w324:refnum<file>)  [unwired: 4 in, 2 out]
      n106 = Unbundle(w331) -> ("Velocity (fps)"=w329:dbl, "Accel (fps^2)"=w328:dbl, "Jerk (fps^3)"=w327:dbl, "StoopidFast (fps)"=w326:dbl)
      n107 = Bundle("Velocity (fps)"=w329, "Accel (fps^2)"=w328, "Jerk (fps^3)"=w327, "StoopidFast (fps)"=w326) -> (w330:T30)  [unwired: 1 in]
      n108 = Read from Binary File(5:FALSE, 11:w324) -> (2:w322:bool, 3:w317:refnum<file>)  [unwired: 4 in, 2 out]
      n109 = Read from Binary File(5:cluster{"Drive Type":T3, "Path Type":T4} {"Drive Type"=enum."Nonholonomic", "Path Type"=enum."Clothoid"} ("Trajectory Meta"), 11:w317) -> (2:w314:cluster{"Drive Type":T3, "Path Type":T4}, 3:w315:refnum<file>)  [unwired: 4 in, 2 out]
    }
  }
  "Zero V" <- w19
  "Reversals" <- w18
  "Commands out" <- w16
  "Points out" <- w14
  "Overall" <- w5
  "Trajectory Meta" <- w1
  "Trajectory Data" <- w13
  n110 = Bundle("Sample Period (s)"=w21, w22, "Conditions"=w23, "Overrides"=w24, "Angular Limits"=w2) -> (→"Fields":T7)  [unwired: 1 in]
  n111 = Close File(refnum=w10) -> ()  [unwired: 1 in, 2 out]
